vi "G-Class_Ref.vi"(7 "枚举":enum16{"R", "W"}(ring), 10 "句柄输入":refnum<class "G-Uart-Class.lvclass">) -> (2 "句柄输出":refnum<class "G-Uart-Class.lvclass">)   [LabVIEW 2025, in "G-Uart-Class.lvclass"]
uses:
  G-Uart-Class.lvclass
panel:
  # "这个句柄是为了方便别的地方调用\n但是这违反了低耦合高内聚\n属于要适应程序的无奈之举\n不要使用这个vi"
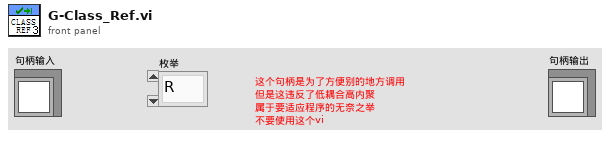
[diagram p1: front panel]
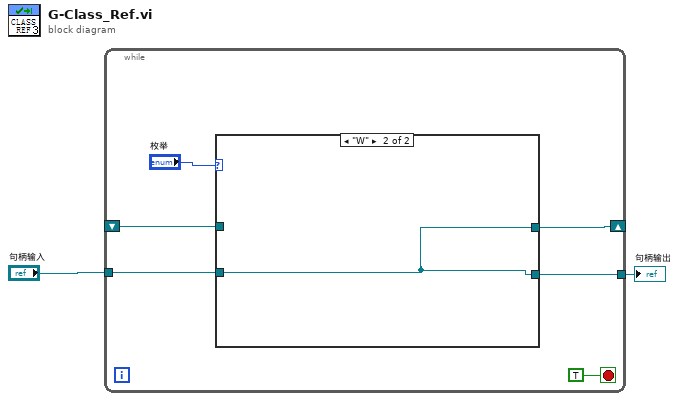
[diagram p0: block diagram]
diagram:
  n1 = while {
    shift-right: [w6] -> _
    shift-left: _ -> [w4]
    tunnel: "句柄输入" -> [w5]
    tunnel: [w3] -> w1
    stop <- TRUE stop-if-true
    n2 = case shown="\"W\"" "枚举" {
      tunnel: [w9 w10] -> w6
      tunnel: w5 -> [_ w10]
      tunnel: w4 -> [w9 _]
      tunnel: [w9 w10] -> w3
      frame "R", Default {
      }
      frame "W" {
      }
    }
  }
  "句柄输出" <- w1
